vi "Target_Main.vi"(8 "error in (no error)":errorcluster={"status"=FALSE, "code"=0, "source"="\"\""}, 10 "hardware/transport profile":string="PROFILE_DEFAULT", 11 "Local paths":string="C:\\Config") -> (0 "error out":errorcluster={"status"=FALSE, "code"=0, "source"="\"\""}, 2 "status ok":bool, 3 "Shutdown/status":string)   [LabVIEW 2026]
doc: "INTENT: Top-level cRIO/RT Target Executive initializing services, executing supervisory loop, and closing cleanly."
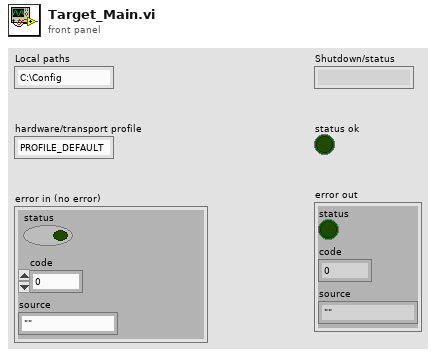
[diagram p1: front panel]
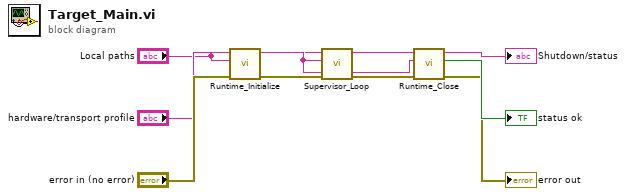
[diagram p0: block diagram]
diagram:
  n1 = call "Runtime_Initialize.vi"("error in (no error)"="error in (no error)", "configuration locations"="Local paths", "Target capability"="hardware/transport profile") -> ("error out"=w5:errorcluster, "Service references"=w4:string)  [unwired: 6 in, 1 out]
  n2 = call "Supervisor_Loop.vi"("error in (no error)"=w5, "RunContext"=w4, "Supervisor message queue"="Local paths") -> ("error out"=w7:errorcluster, "State transitions/events"=w6:string)  [unwired: 6 in, 1 out]
  n3 = call "Runtime_Close.vi"("error in (no error)"=w7, "service references"=w4, "Run state"=w6) -> ("error out"=→"error out":errorcluster, "status ok"=→"status ok":bool, "Close results"=→"Shutdown/status":string)  [unwired: 6 in]
